vi "SeqEditor.vi"(8 "error in (no error)":errorcluster, 11 "NLTest in":refnum<class "NLTest.lvclass">) -> (0 "error out":errorcluster, 3 "NLTest out":refnum<class "NLTest.lvclass">)   [LabVIEW 2017, in "NLTest.lvclass"]
uses:
  NLTest.lvclass
  seqeditor-rollbackbtn.ctl
  seqeditor-reloadDEFstepbtn.ctl
  NLTest.lvclass/NLTest.ctl
  SeqEditor_Global.vi
panel:
  in  "ReNameBox":string
  in  "VarTableVISA":refnum<visa-resource-name>
  in  "VarTablePath":path
  in  "VarTableFxEnumC":u16(ring) caption="2147483647" items=["-", "Set Default!", "-", "New var"]
  in  "VarTableFx":string
  in  "重载":T1
  in  "已复制":bool
  in  "Rollback":T2
  in  "内部拖拽":bool
  in  "Param集":i32(listbox)
  in  "步骤原型":i32(listbox)
  in  "Step集":i32[](listbox)
  in  "序列总表":i32(listbox)
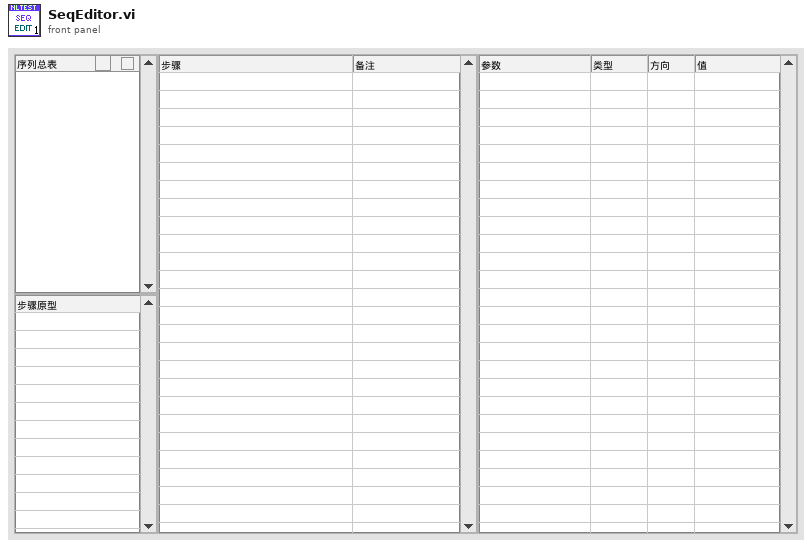
[diagram p1: front panel]
types:
  T1 = typedef "NLTest.lvclass/seqeditor-reloadDEFstepbtn.ctl" = bool
  T2 = typedef "NLTest.lvclass/seqeditor-rollbackbtn.ctl" = bool
  T3 = typedef "LVPoint32TypeDef.ctl" = cluster{"Horizontal":i32, "Vertical":i32}
  T4 = typedef "eventvkey.ctl" = enum16{"ASCII", "Enter", "Return", "Shift", "Ctrl", "Alt", "Cmd", "Opt", "Caps", "NumLock", "Clear", "Break", "Up", "Down", "Left", "Right", "Insert", "Delete", "Home", "End", "PageUp", "PageDown", "Escape", "Help", "Pause", "ScrollLock", "F1", "F2", "F3", "F4", "F5", "F6", "F7", "F8", "F9", "F10", "F11", "F12", "F13", "F14", "F15", "F16", "F17", "F18", "F19", "F20", "F21", "F22", "F23", "F24", "Play", "VolumeUp", "VolumeDown", "Mute", "Two Byte Char"}
  T5 = enum16{"Left Button", "Center Button", "Right Button", "Window Close"}
  T6 = enum32{"Invalid", "Standard", "Closed", "Hidden", "Minimized", "Maximized"}
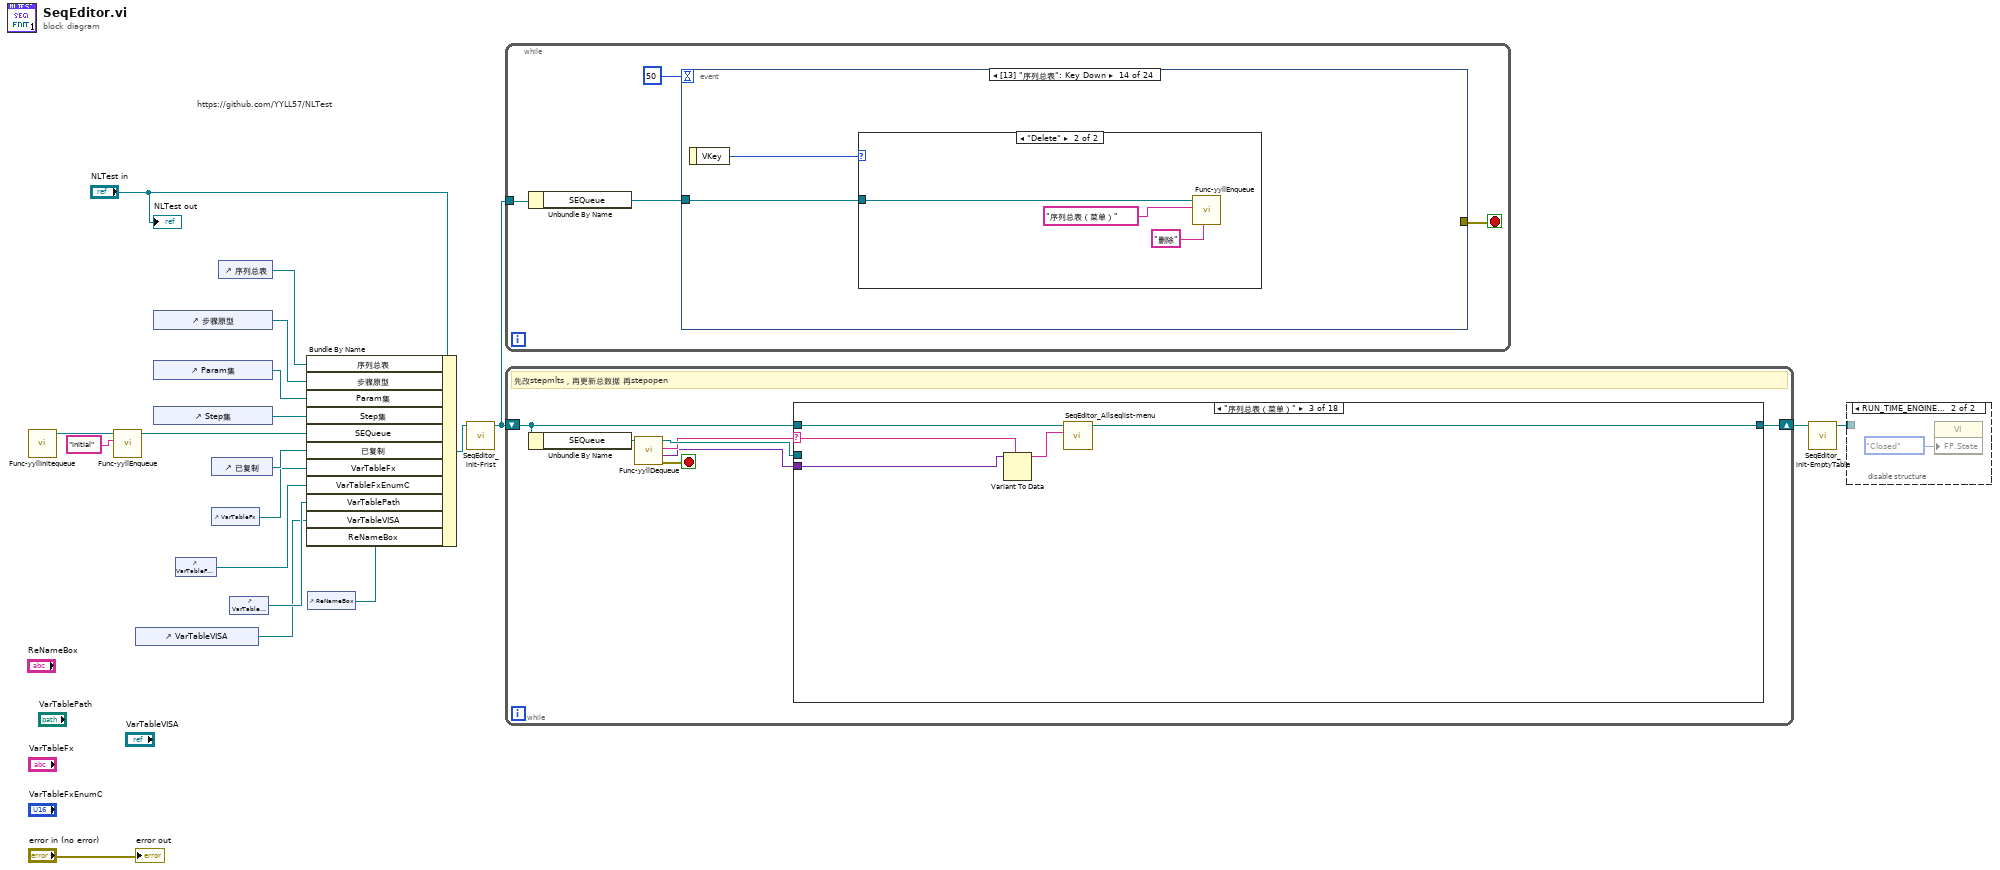
[diagram p0: block diagram]
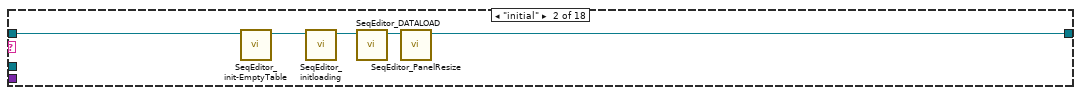
[diagram p4: hidden frame]
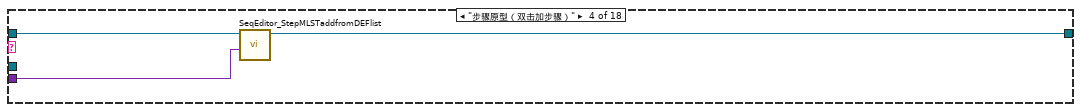
[diagram p5: hidden frame]
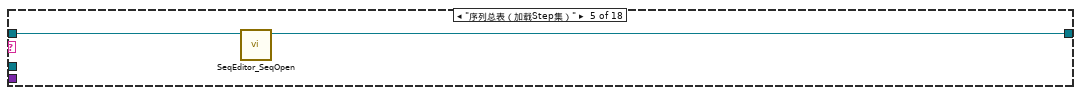
[diagram p6: hidden frame]
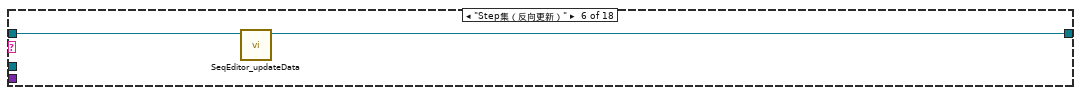
[diagram p7: hidden frame]
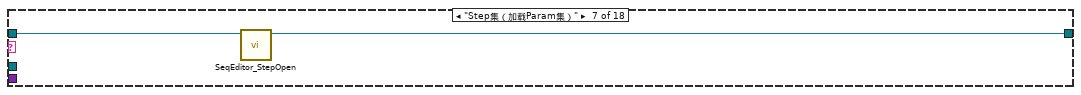
[diagram p8: hidden frame]
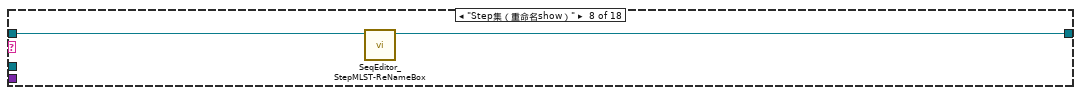
[diagram p9: hidden frame]
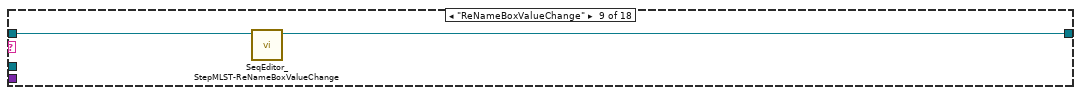
[diagram p10: hidden frame]
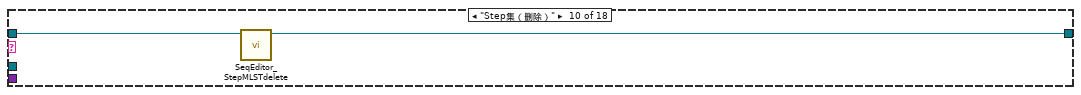
[diagram p11: hidden frame]
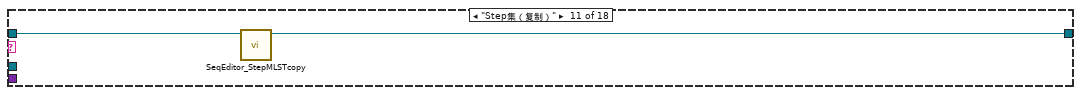
[diagram p12: hidden frame]
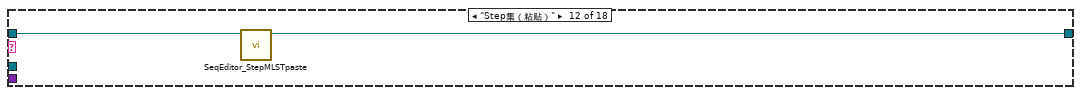
[diagram p13: hidden frame]
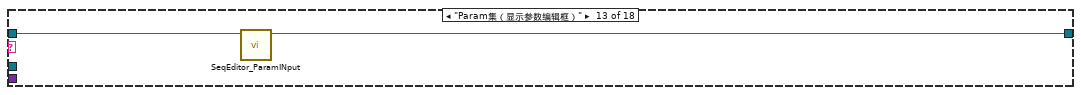
[diagram p14: hidden frame]
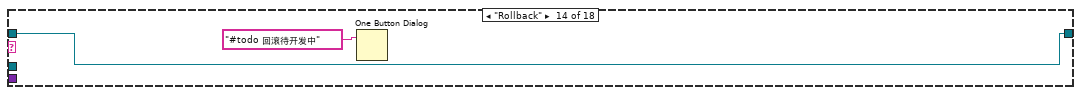
[diagram p15: hidden frame]
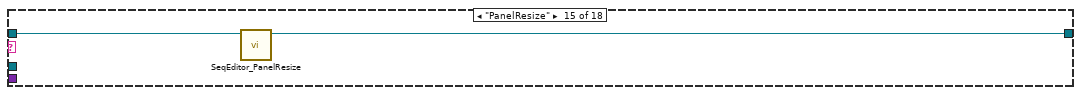
[diagram p16: hidden frame]
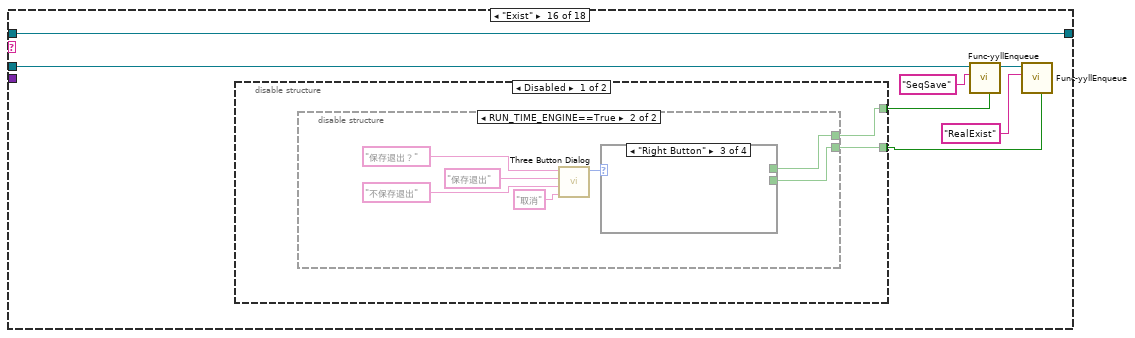
[diagram p17: hidden frame]
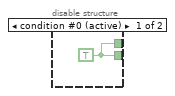
[diagram p18: hidden frame]
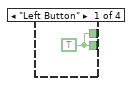
[diagram p19: hidden frame]
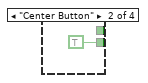
[diagram p20: hidden frame]
diagram:
  # "https://github.com/YYLL57/NLTest"
  n1 = call "Func-yyllInitequeue.vi"() -> ("queue out"=w18:refnum<queue>)  [unwired: 8 in, 3 out]
  n2 = call "Func-yyllEnqueue.vi"("cmd"="initial", "queue in"=w18) -> ("queue out"=w12:refnum<queue>)  [unwired: 7 in, 2 out]
  n3 = control-ref of="VarTableVISA"() -> (w2:refnum<vi>)
  n4 = control-ref of="步骤原型"() -> (w16:refnum<vi>)
  n5 = control-ref of="Param集"() -> (w15:refnum<vi>)
  n6 = control-ref of="Step集"() -> (w14:refnum<vi>)
  n7 = control-ref of="VarTableFxEnumC"() -> (w4:refnum<vi>)
  n8 = control-ref of="已复制"() -> (w8:refnum<vi>)
  n9 = control-ref of="VarTableFx"() -> (w5:refnum<vi>)
  n10 = control-ref of="序列总表"() -> (w13:refnum<vi>)
  n11 = control-ref of="VarTablePath"() -> (w3:refnum<vi>)
  n12 = control-ref of="ReNameBox"() -> (w1:refnum<vi>)
  n13 = Bundle By Name(cluster="NLTest in", "序列总表"=w13, "步骤原型"=w16, "Param集"=w15, "Step集"=w14, "SEQueue"=w12, "已复制"=w8, "VarTableFx"=w5, "VarTableFxEnumC"=w4, "VarTablePath"=w3, "VarTableVISA"=w2, "ReNameBox"=w1) -> (w7:refnum<class "NLTest.lvclass">)
  n14 = call "SeqEditor_init-Frist.vi"("NLTest in"=w7) -> ("NLTest out"=w6:refnum<class "NLTest.lvclass">)  [unwired: 9 in, 1 out]
  n15 = while {
    tunnel: w6 -> [w21]
    stop <- w22 stop-if-true
    n16 = Unbundle By Name(w21) -> ("SEQueue"=w20:refnum<queue>)
    n17 = event shown="[13] \"序列总表\": Key Down" {
      selector: _ -> [_ _ _ _ _ _ _ _ _ _ _ _ _ _ _ _ _ _ _ _ _ _ _ _]
      dyn-events: _ -> [_ _ _ _ _ _ _ _ _ _ _ _ _ _ _ _ _ _ _ _ _ _ _ _]
      timeout: 50 -> [_ _ _ _ _ _ _ _ _ _ _ _ _ _ _ _ _ _ _ _ _ _ _ _]
      tunnel: [_ _ _ _ _ _ _ _ _ _ _ _ _ _ _ _ _ _ _ _ _ _ _ w111] -> w22
      tunnel: w20 -> [_ w31 w32 _ w48 w56 w64 _ w71 _ w75 _ w81 w85 _ w95 w97 w99 _ w103 w104 w106 w109 w112]
      event "Step集": Drag Starting {
        n18 = event-data() -> ()  [unwired: 1 in, 5 out]
        n19 = local write "内部拖拽"(TRUE ("内部拖拽")) -> ()
      }
      event "Step集": Drop {
        n20 = event-data() -> ("CtlRef"=w29:refnum<vi>, "Coords"=w28:T3, "PlatMods.Ctrl"=w27:bool)  [unwired: 1 in]
        n21 = call "SeqEditor_StepMLSTDrop.vi"("内部拖拽"="内部拖拽", "Ctrl"=w27, "Coords"=w28, "CtlRef"=w29) -> ("error out"=w26:errorcluster)  [unwired: 6 in, 1 out]
        n22 = call "Func-yyllEnqueue.vi"("error in (no error)"=w26, "cmd"="Step集（反向更新）", "queue in"=w31) -> ()  [unwired: 6 in, 3 out]
        n23 = event-data() -> ()  [unwired: 2 in, 1 out]
      }
      event "Step集": Key Up {
        n24 = event-data() -> ("ScanCode"=w33:i16, "PlatMods.Ctrl"=w34:bool)  [unwired: 1 in]
        n25 = case shown="True" w34 {
          tunnel: w33 -> [w36 w40]
          tunnel: w32 -> [w35 w39]
          frame False {
            n26 = case shown="83" w36 {
              tunnel: w35 -> [_ w37]
              frame 0, Default {
              }
              frame 83 {
                n27 = call "Func-yyllEnqueue.vi"("cmd"="Step集（删除）", "queue in"=w37) -> ()  [unwired: 7 in, 3 out]
              }
            }
          }
          frame True {
            n28 = case shown="47" w40 {
              tunnel: w39 -> [_ w41 w43]
              frame 0, Default {
              }
              frame 46 {
                # "ctrl c"
                n29 = call "Func-yyllEnqueue.vi"("cmd"="Step集（复制）", "queue in"=w41) -> ()  [unwired: 7 in, 3 out]
              }
              frame 47 {
                # "ctrl v"
                n30 = call "Func-yyllEnqueue.vi"("cmd"="Step集（粘贴）", "queue in"=w43) -> ()  [unwired: 7 in, 3 out]
              }
            }
          }
        }
      }
      event "Step集": Shortcut Menu Activation? {
        n31 = event-data() -> ("MenuRef"=w47:refnum<k9>)  [unwired: 1 in, 5 out]
        n32 = Delete Menu Items(9:w47) -> (3:w46:refnum<k9>)  [unwired: 3 in, 1 out]
        n33 = Insert Menu Items(7:string[] ["复制", "粘贴", "删除"] ("item tags"), 9:w46) -> ()  [unwired: 4 in, 3 out]
        n34 = event-data() -> ()  [unwired: 2 in, 1 out]
      }
      event "Step集": Shortcut Menu Selection (User) {
        n35 = event-data() -> ("ItemTag"=w49:string)  [unwired: 1 in, 5 out]
        n36 = case shown="\"粘贴\"" w49 {
          tunnel: w48 -> [_ w51 w53 w55]
          frame "False", Default {
          }
          frame "删除" {
            n37 = call "Func-yyllEnqueue.vi"("cmd"="Step集（删除）", "queue in"=w51) -> ()  [unwired: 7 in, 3 out]
          }
          frame "复制" {
            n38 = call "Func-yyllEnqueue.vi"("cmd"="Step集（复制）", "queue in"=w53) -> ()  [unwired: 7 in, 3 out]
          }
          frame "粘贴" {
            n39 = call "Func-yyllEnqueue.vi"("cmd"="Step集（粘贴）", "queue in"=w55) -> ()  [unwired: 7 in, 3 out]
          }
        }
      }
      event "Step集": Value Change {
        n40 = event-data() -> ()  [unwired: 1 in, 2 out]
        n41 = call "Func-yyllEnqueue.vi"("cmd"="Step集（加载Param集）", "queue in"=w56) -> ()  [unwired: 7 in, 3 out]
      }
      event "Step集": Mouse Up {
        n42 = event-data() -> ("CtlRef"=w65:refnum<vi>)  [unwired: 1 in, 5 out]
        n43 = property class="MCListbox (strict)"(reference=w65) -> (reference out=w63:refnum<vi>, "ItemNames"=w62:string[][])  [unwired: 1 in, 1 out]
        n44 = Matrix Size(0:w62) -> (1:w61:i32)  [unwired: 1 out]
        n45 = invoke class="MCListbox (strict)" method="Get DblClk Row"(reference=w63) -> ("Get Double-clicked Row"=w58:i32)  [unwired: 2 in, 2 out]
        n46 = In Range and Coerce(upper limit=w61, x=w58, lower limit=0) -> (In Range?=w59:bool)  [unwired: 1 out]
        n47 = case shown="True" w59 {
          tunnel: w64 -> [_ w67]
          tunnel: w58 -> [_ w66]
          frame False {
          }
          frame True {
            n48 = global write "SeqEditor_Global.vi" "Step集选择行"(w66) -> ()
            n49 = call "Func-yyllEnqueue.vi"("cmd"="Step集（重命名show）", "queue in"=w67) -> ()  [unwired: 7 in, 3 out]
          }
        }
      }
      event "ReNameBox": Mouse Leave {
        n50 = event-data() -> ("CtlRef"=w70:refnum<vi>)  [unwired: 1 in, 3 out]
        n51 = property class="Str"(reference=w70, "Visible"=FALSE) -> ()  [unwired: 1 in, 2 out]
      }
      event "ReNameBox": Value Change {
        n52 = event-data() -> ()  [unwired: 1 in, 6 out]
        n53 = call "Func-yyllEnqueue.vi"("cmd"="ReNameBoxValueChange", "queue in"=w71) -> ()  [unwired: 7 in, 3 out]
      }
      event "步骤原型": Drag Starting {
        n54 = event-data() -> ()  [unwired: 1 in, 5 out]
        n55 = local write "内部拖拽"(FALSE ("内部拖拽")) -> ()
      }
      event "步骤原型": Mouse Up {
        n56 = event-data() -> ("CtlRef"=w77:refnum<vi>)  [unwired: 1 in]
        n57 = invoke class="MCListbox (strict)" method="Get DblClk Row"(reference=w77) -> ("Get Double-clicked Row"=w74:i32)  [unwired: 2 in, 2 out]
        n58 = call "Func-yyllEnqueue.vi"("data"=w74, "cmd"="步骤原型（双击加步骤）", "queue in"=w75) -> ()  [unwired: 6 in, 3 out]
      }
      event "步骤原型": Shortcut Menu Activation? {
        n59 = event-data() -> ("MenuRef"=w80:refnum<k9>)  [unwired: 1 in, 5 out]
        n60 = Delete Menu Items(9:w80) -> (3:w79:refnum<k9>)  [unwired: 3 in, 1 out]
        n61 = Insert Menu Items(7:string[] ["重载"] ("item tags"), 9:w79) -> ()  [unwired: 4 in, 3 out]
        n62 = event-data() -> ()  [unwired: 2 in, 1 out]
      }
      event "步骤原型": Shortcut Menu Selection (User) {
        n63 = event-data() -> ("ItemTag"=w82:string)  [unwired: 1 in]
        n64 = case shown="\"重载\"" w82 {
          tunnel: w81 -> [_ w84]
          frame "False", Default {
          }
          frame "重载" {
            n65 = call "Func-yyllEnqueue.vi"("cmd"="initial", "queue in"=w84) -> ()  [unwired: 7 in, 3 out]
          }
        }
      }
      event "序列总表": Key Down {
        n66 = event-data() -> ("VKey"=w86:T4)  [unwired: 1 in]
        n67 = case shown="\"Delete\"" w86 {
          tunnel: w85 -> [_ w89]
          frame "ASCII", Default {
          }
          frame "Delete" {
            n68 = call "Func-yyllEnqueue.vi"("data"="删除", "cmd"="序列总表（菜单）", "queue in"=w89) -> ()  [unwired: 6 in, 3 out]
          }
        }
      }
      event "序列总表": Shortcut Menu Activation? {
        n69 = event-data() -> ("MenuRef"=w92:refnum<k9>)  [unwired: 1 in]
        n70 = Delete Menu Items(9:w92) -> (3:w91:refnum<k9>)  [unwired: 3 in, 1 out]
        n71 = Insert Menu Items(7:string[] ["新建", "删除", "复制", "重命名", "帮助"] ("item tags"), 9:w91) -> ()  [unwired: 4 in, 3 out]
        n72 = event-data() -> ()  [unwired: 2 in, 1 out]
      }
      event "序列总表": Shortcut Menu Selection (User) {
        n73 = event-data() -> ("ItemTag"=w94:string)  [unwired: 1 in]
        n74 = call "Func-yyllEnqueue.vi"("data"=w94, "cmd"="序列总表（菜单）", "queue in"=w95) -> ()  [unwired: 6 in, 3 out]
      }
      event "序列总表": Value Change {
        n75 = event-data() -> ()  [unwired: 1 in, 6 out]
        n76 = call "Func-yyllEnqueue.vi"("cmd"="序列总表（加载Step集）", "queue in"=w97) -> ()  [unwired: 7 in, 3 out]
      }
      event "Param集": Value Change {
        n77 = event-data() -> ()  [unwired: 1 in, 6 out]
        n78 = call "Func-yyllEnqueue.vi"("cmd"="Param集（显示参数编辑框）", "queue in"=w99) -> ()  [unwired: 7 in, 3 out]
      }
      event "Param集": Mouse Down {
        n79 = event-data() -> ("CtlRef"=w101:refnum<vi>, "Coords"=w100:T3)  [unwired: 1 in]
        n80 = call "SeqEditor_ParamMousehit.vi"("Coords"=w100, "MulticolumnListbox in"=w101) -> ()  [unwired: 10 in]
      }
      event Value Change {
        n81 = event-data() -> ()  [unwired: 1 in, 6 out]
        n82 = call "Func-yyllEnqueue.vi"("cmd"="Rollback", "queue in"=w103) -> ()  [unwired: 7 in, 3 out]
      }
      event Value Change {
        n83 = event-data() -> ()  [unwired: 1 in, 6 out]
        n84 = call "Func-yyllEnqueue.vi"("cmd"="initial", "queue in"=w104) -> ()  [unwired: 7 in, 3 out]
      }
      event Panel Close? {
        n85 = event-data() -> ()  [unwired: 1 in, 1 out]
        n86 = call "Func-yyllEnqueue.vi"("cmd"="Exist", "queue in"=w106) -> ()  [unwired: 7 in, 3 out]
        n87 = event-data("Discard?"=TRUE) -> ()  [unwired: 1 in, 1 out]
      }
      event Panel Resize {
        n88 = event-data() -> ()  [unwired: 1 in, 6 out]
        n89 = call "Func-yyllEnqueue.vi"("cmd"="PanelResize", "queue in"=w109) -> ()  [unwired: 7 in, 3 out]
      }
      event Timeout {
        n90 = event-data() -> ()  [unwired: 1 in, 1 out]
        n91 = Get Queue Status(queue=w112) -> (error out=w111:errorcluster)  [unwired: 2 in, 7 out]
      }
    }
  }
  n92 = while {
    shift-right: [w115] -> w10
    shift-left: w6 -> [w114]
    stop <- w118 stop-if-true
    # "先改stepmlts，再更新总数据 再stepopen"
    n93 = Unbundle By Name(w114) -> ("SEQueue"=w113:refnum<queue>)
    n94 = call "Func-yyllDequeue.vi"("queue in"=w113) -> ("error out"=w118:errorcluster, "data"=w116:variant, "cmd"=w117:string, "queue out"=w119:refnum<queue>)  [unwired: 6 in, 1 out]
    n95 = case shown="\"序列总表（菜单）\"" w117 {
      selector: w117 -> [_ _ w127 _ _ _ _ _ _ _ _ _ _ _ _ _ _ _]
      tunnel: w119 -> [_ _ _ _ _ _ _ _ _ _ _ _ _ _ _ w160 _ w179]
      tunnel: w116 -> [_ _ w128 w131 _ _ _ _ _ _ _ _ _ _ _ _ _ _]
      tunnel: w114 -> [w120 w125 w129 w132 w135 w136 w139 w140 w142 w144 w146 w148 w150 w153 w154 w156 w176 w178]
      tunnel: [w120 w122 w130 w133 w134 w137 w138 w141 w143 w145 w147 w149 w151 w153 w155 w156 w177 w178] -> w115
      frame "idle", Default {
      }
      frame "initial" {
        n96 = call "SeqEditor_init-EmptyTable.vi"("NLTest in"=w125) -> ("NLTest out"=w123:refnum<class "NLTest.lvclass">)  [unwired: 9 in, 1 out]
        n97 = call "SeqEditor_initloading.vi"("NLTest in"=w123) -> ("NLTest out"=w124:refnum<class "NLTest.lvclass">)  [unwired: 9 in, 1 out]
        n98 = call "SeqEditor_DATALOAD.vi"("NLTest in"=w124) -> ("NLTest out"=w121:refnum<class "NLTest.lvclass">)  [unwired: 9 in, 1 out]
        n99 = call "SeqEditor_PanelResize.vi"("NLTest in"=w121) -> ("NLTest out"=w122:refnum<class "NLTest.lvclass">)  [unwired: 9 in, 1 out]
      }
      frame "序列总表（菜单）" {
        n100 = Variant To Data(type=w127, Variant=w128) -> (data=w126:string)  [unwired: 1 in, 1 out]
        n101 = call "SeqEditor_Allseqlist-menu.vi"("String"=w126, "NLTest in"=w129) -> ("NLTest out"=w130:refnum<class "NLTest.lvclass">)  [unwired: 8 in, 1 out]
      }
      frame "步骤原型（双击加步骤）" {
        n102 = call "SeqEditor_StepMLSTaddfromDEFlist.vi"("Double-Clicked Row"=w131, "NLTest in"=w132) -> ("NLTest out"=w133:refnum<class "NLTest.lvclass">)  [unwired: 8 in, 1 out]
      }
      frame "序列总表（加载Step集）" {
        n103 = call "SeqEditor_SeqOpen.vi"("NLTest in"=w135) -> ("NLTest out"=w134:refnum<class "NLTest.lvclass">)  [unwired: 9 in, 1 out]
      }
      frame "Step集（反向更新）" {
        n104 = call "SeqEditor_updateData.vi"("NLTest in"=w136) -> ("NLTest out"=w137:refnum<class "NLTest.lvclass">)  [unwired: 9 in, 1 out]
      }
      frame "Step集（加载Param集）" {
        n105 = call "SeqEditor_StepOpen.vi"("NLTest in"=w139) -> ("NLTest out"=w138:refnum<class "NLTest.lvclass">)  [unwired: 9 in, 1 out]
      }
      frame "Step集（重命名show）" {
        n106 = call "SeqEditor_StepMLST-ReNameBox.vi"("NLTest in"=w140) -> ("NLTest out"=w141:refnum<class "NLTest.lvclass">)  [unwired: 9 in, 1 out]
      }
      frame "ReNameBoxValueChange" {
        n107 = call "SeqEditor_StepMLST-ReNameBoxValueChange.vi"("NLTest in"=w142) -> ("NLTest out"=w143:refnum<class "NLTest.lvclass">)  [unwired: 9 in, 1 out]
      }
      frame "Step集（删除）" {
        n108 = call "SeqEditor_StepMLSTdelete.vi"("NLTest in"=w144) -> ("NLTest out"=w145:refnum<class "NLTest.lvclass">)  [unwired: 9 in, 1 out]
      }
      frame "Step集（复制）" {
        n109 = call "SeqEditor_StepMLSTcopy.vi"("NLTest in"=w146) -> ("NLTest out"=w147:refnum<class "NLTest.lvclass">)  [unwired: 9 in, 1 out]
      }
      frame "Step集（粘贴）" {
        n110 = call "SeqEditor_StepMLSTpaste.vi"("NLTest in"=w148) -> ("NLTest out"=w149:refnum<class "NLTest.lvclass">)  [unwired: 9 in, 1 out]
      }
      frame "Param集（显示参数编辑框）" {
        n111 = call "SeqEditor_ParamINput.vi"("NLTest in"=w150) -> ("NLTest out"=w151:refnum<class "NLTest.lvclass">)  [unwired: 9 in, 1 out]
      }
      frame "Rollback" {
        n112 = One Button Dialog(message="#todo 回滚待开发中") -> ()  [unwired: 1 in, 1 out]
      }
      frame "PanelResize" {
        n113 = call "SeqEditor_PanelResize.vi"("NLTest in"=w154) -> ("NLTest out"=w155:refnum<class "NLTest.lvclass">)  [unwired: 9 in, 1 out]
      }
      frame "Exist" {
        n114 = disable-structure shown="Disabled" {
          disable-tunnel: [w164 w175] -> w158
          disable-tunnel: [w163 w175] -> w157
          frame Disabled {
            n115 = disable-structure shown="RUN_TIME_ENGINE==True" {
              disable-tunnel: [w165 w167] -> w164
              disable-tunnel: [w165 w166] -> w163
              frame condition #0 (active) {
                w165 = TRUE ("Enable?(T)")
              }
              frame condition #1 {
                n116 = call <vilib>:"Three Button Dialog.vi"("Right Button Text (\"Cancel\")"="取消" ("Center Button Text (\"No\")"), "Center Button Text (\"No\")"="不保存退出" ("Center Button Text (\"No\")"), "Left Button Text (\"Yes\")"="保存退出" ("Left Button Text (\"Yes\")"), "message"="保存退出？") -> ("Which Button?"=w172:T5)  [unwired: 7 in]
                n117 = case shown="\"Right Button\"" w172 {
                  tunnel: [w173 _ _ _] -> w167
                  tunnel: [w173 TRUE _ _] -> w166
                  frame "Left Button" {
                    w173 = TRUE
                  }
                  frame "Center Button" {
                  }
                  frame "Right Button" {
                  }
                  frame "Window Close" {
                  }
                }
              }
            }
          }
          frame Enabled {
            w175 = TRUE
          }
        }
        n118 = call "Func-yyllEnqueue.vi"("Enable?(T)"=w158, "cmd"="SeqSave", "queue in"=w160) -> ("queue out"=w161:refnum<queue>)  [unwired: 6 in, 2 out]
        n119 = call "Func-yyllEnqueue.vi"("Enable?(T)"=w157, "cmd"="RealExist", "queue in"=w161) -> ()  [unwired: 6 in, 3 out]
      }
      frame "SeqSave" {
        n120 = call "SeqEditor_DATASAVE.vi"("NLTest in"=w176) -> ("NLTest out"=w177:refnum<class "NLTest.lvclass">)  [unwired: 9 in, 1 out]
      }
      frame "RealExist" {
        n121 = Release Queue(queue=w179, force destroy? (F)=TRUE) -> ()  [unwired: 1 in, 3 out]
      }
    }
  }
  n122 = call "SeqEditor_init-EmptyTable.vi"("NLTest in"=w10) -> ("NLTest out"=w9:refnum<class "NLTest.lvclass">)  [unwired: 9 in, 1 out]
  n123 = disable-structure shown="RUN_TIME_ENGINE==True" {
    disable-tunnel: w9 -> [_ _]
    frame condition #0 (active) {
    }
    frame condition #1 {
      n124 = property class="VI"("FP.State"=T6."Closed" ("前面板窗口:状态")) -> ()  [unwired: 2 in, 2 out]
    }
  }
  "error out" <- "error in (no error)"
  "NLTest out" <- "NLTest in"
